vi "ProjG.vi"(8 "error in":errorcluster) -> (0 "error out":errorcluster)   [LabVIEW 2025]
uses:
  Enum(ctrl1).ctl
  Cluster(ctrl2).ctl
  Ldbrd_cl(ctrl3).ctl
  f9678b56-3cec-4690-80ba-5264990e7274.vi
  <vilib>/Array/Sort 2D Array - Pop Stack.vi
  <vilib>/Array/Sort 2D Array - Push Stack.vi
  <vilib>/Utility/file.llb/Read Delimited Spreadsheet (string).vi
  <vilib>/Instr/_visa.llb/VISA Configure Serial Port (Instr).vi
  <vilib>/Utility/file.llb/Write Delimited Spreadsheet (string).vi
  <vilib>/Analysis/NI_AAL_SigProc.lvlib
  <vilib>/ptbypt/NI_PtbyPt.lvlib
panel:
  in  "stop":bool
  out "LeaderBoard":string[][](array[string])
  in  "VISA port":refnum<visa-resource-name>
  out "HR":cluster{i32[], i32[]}(graph)
  out "Live HR":i32(graph)
  in  "Ldbrd":bool
  in  "Save":bool
  in  "Play":bool
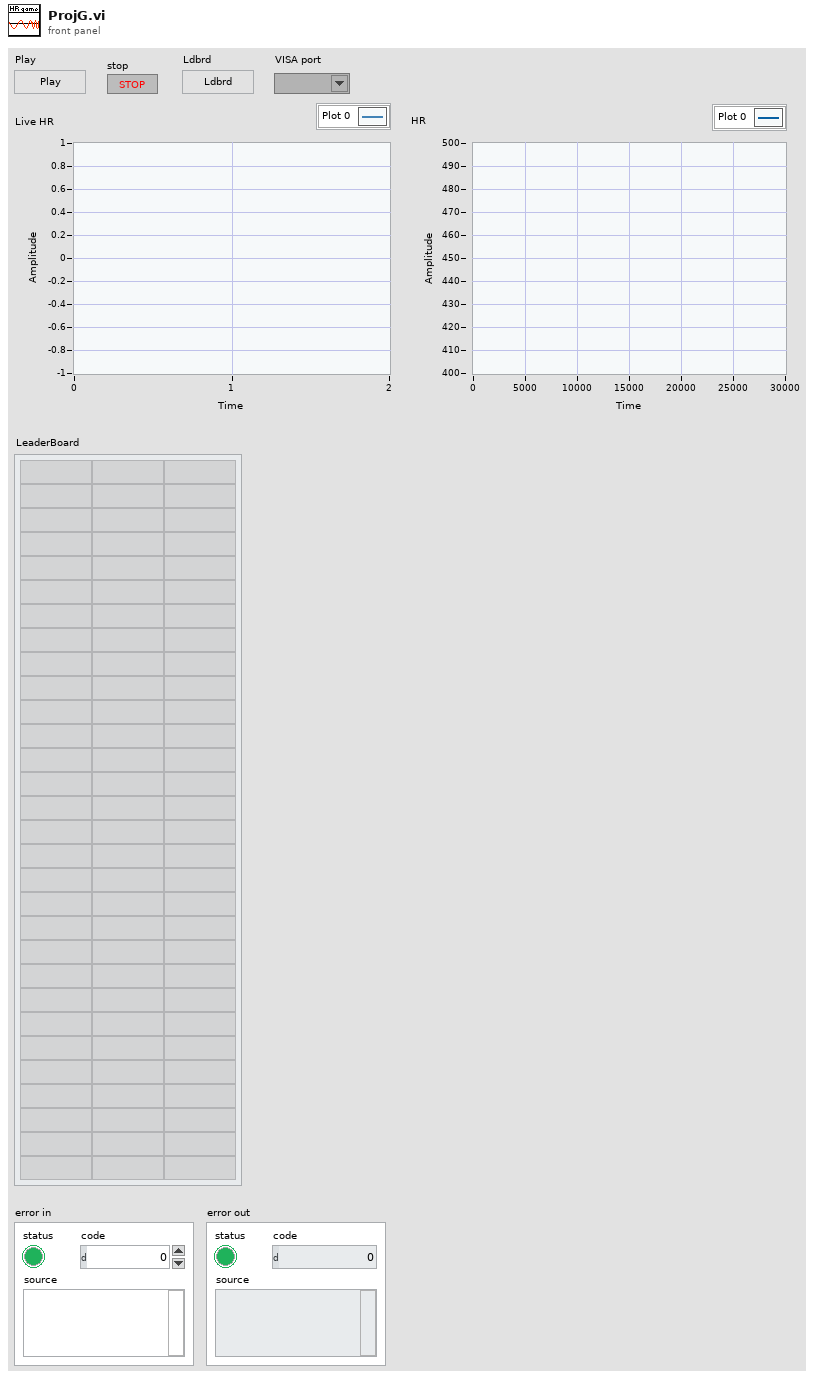
[diagram p1: front panel]
types:
  T1 = typedef "Ldbrd_cl(ctrl3).ctl" = cluster{"Ldbrd":string[][]}
  T2 = typedef "Cluster(ctrl2).ctl" = cluster{"Max HR":i8, "Name":string, "Avg HR":i8}
  T3 = typedef "Enum(ctrl1).ctl" = enum16{"Idle", "Init", "Play", "Ldbrd", "Display", "Save"}
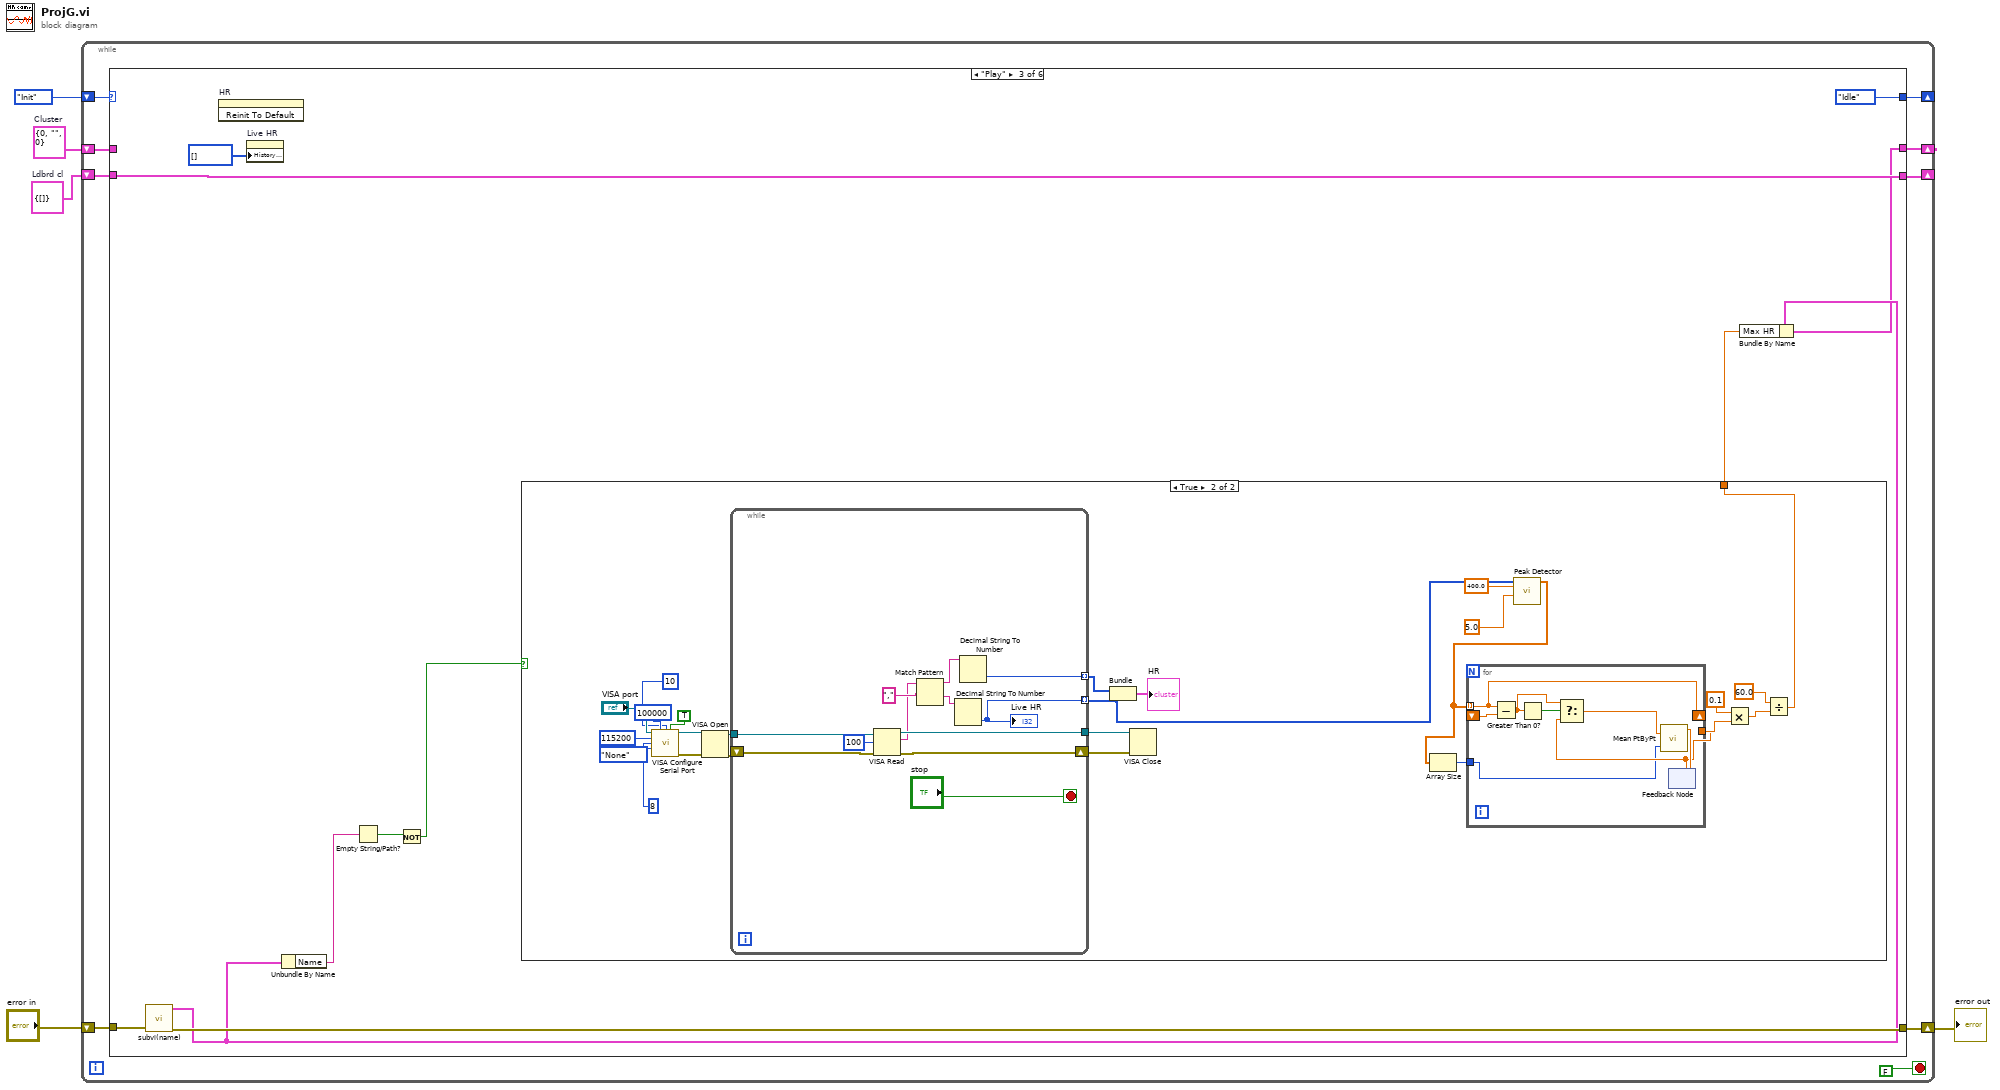
[diagram p0: block diagram]
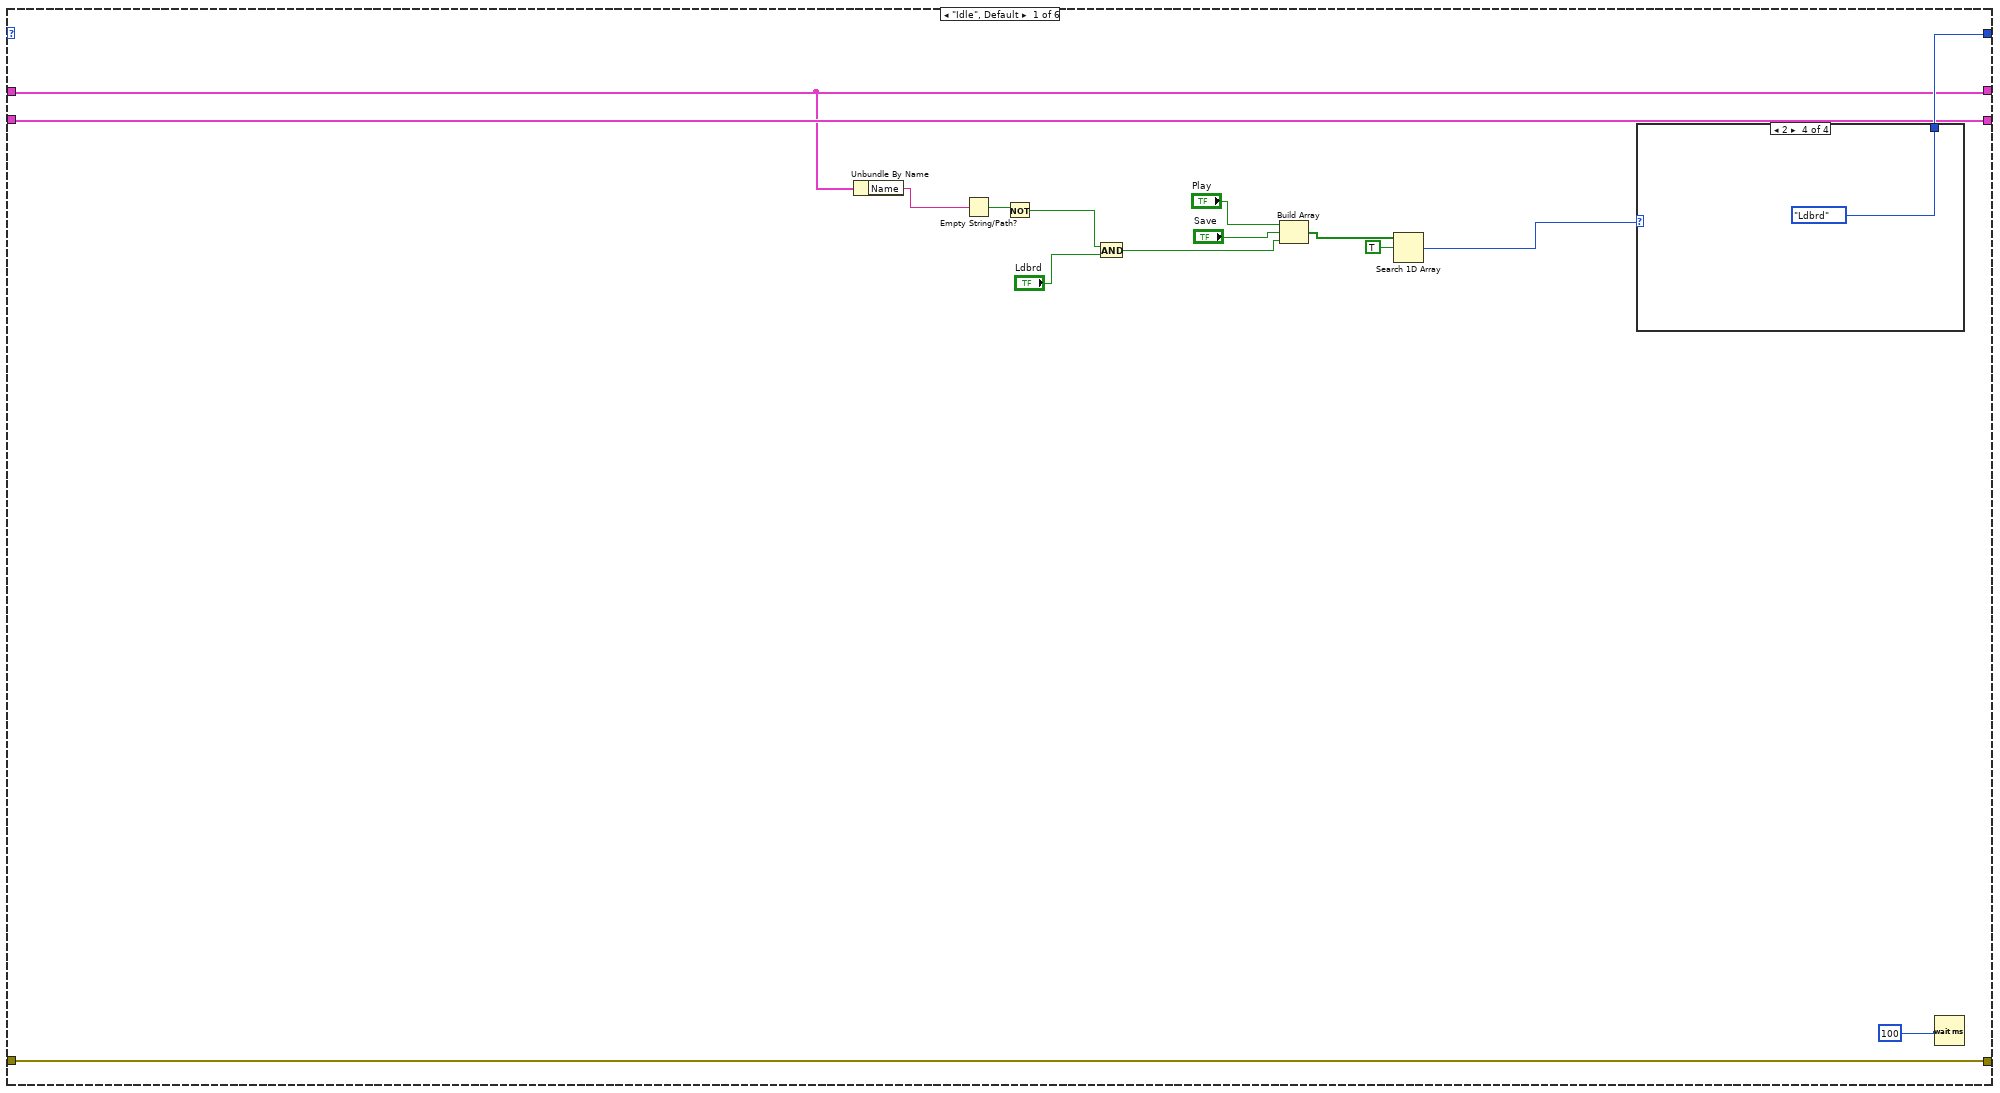
[diagram p2: hidden frame]
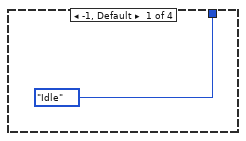
[diagram p3: hidden frame]
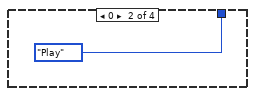
[diagram p4: hidden frame]
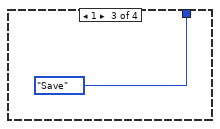
[diagram p5: hidden frame]
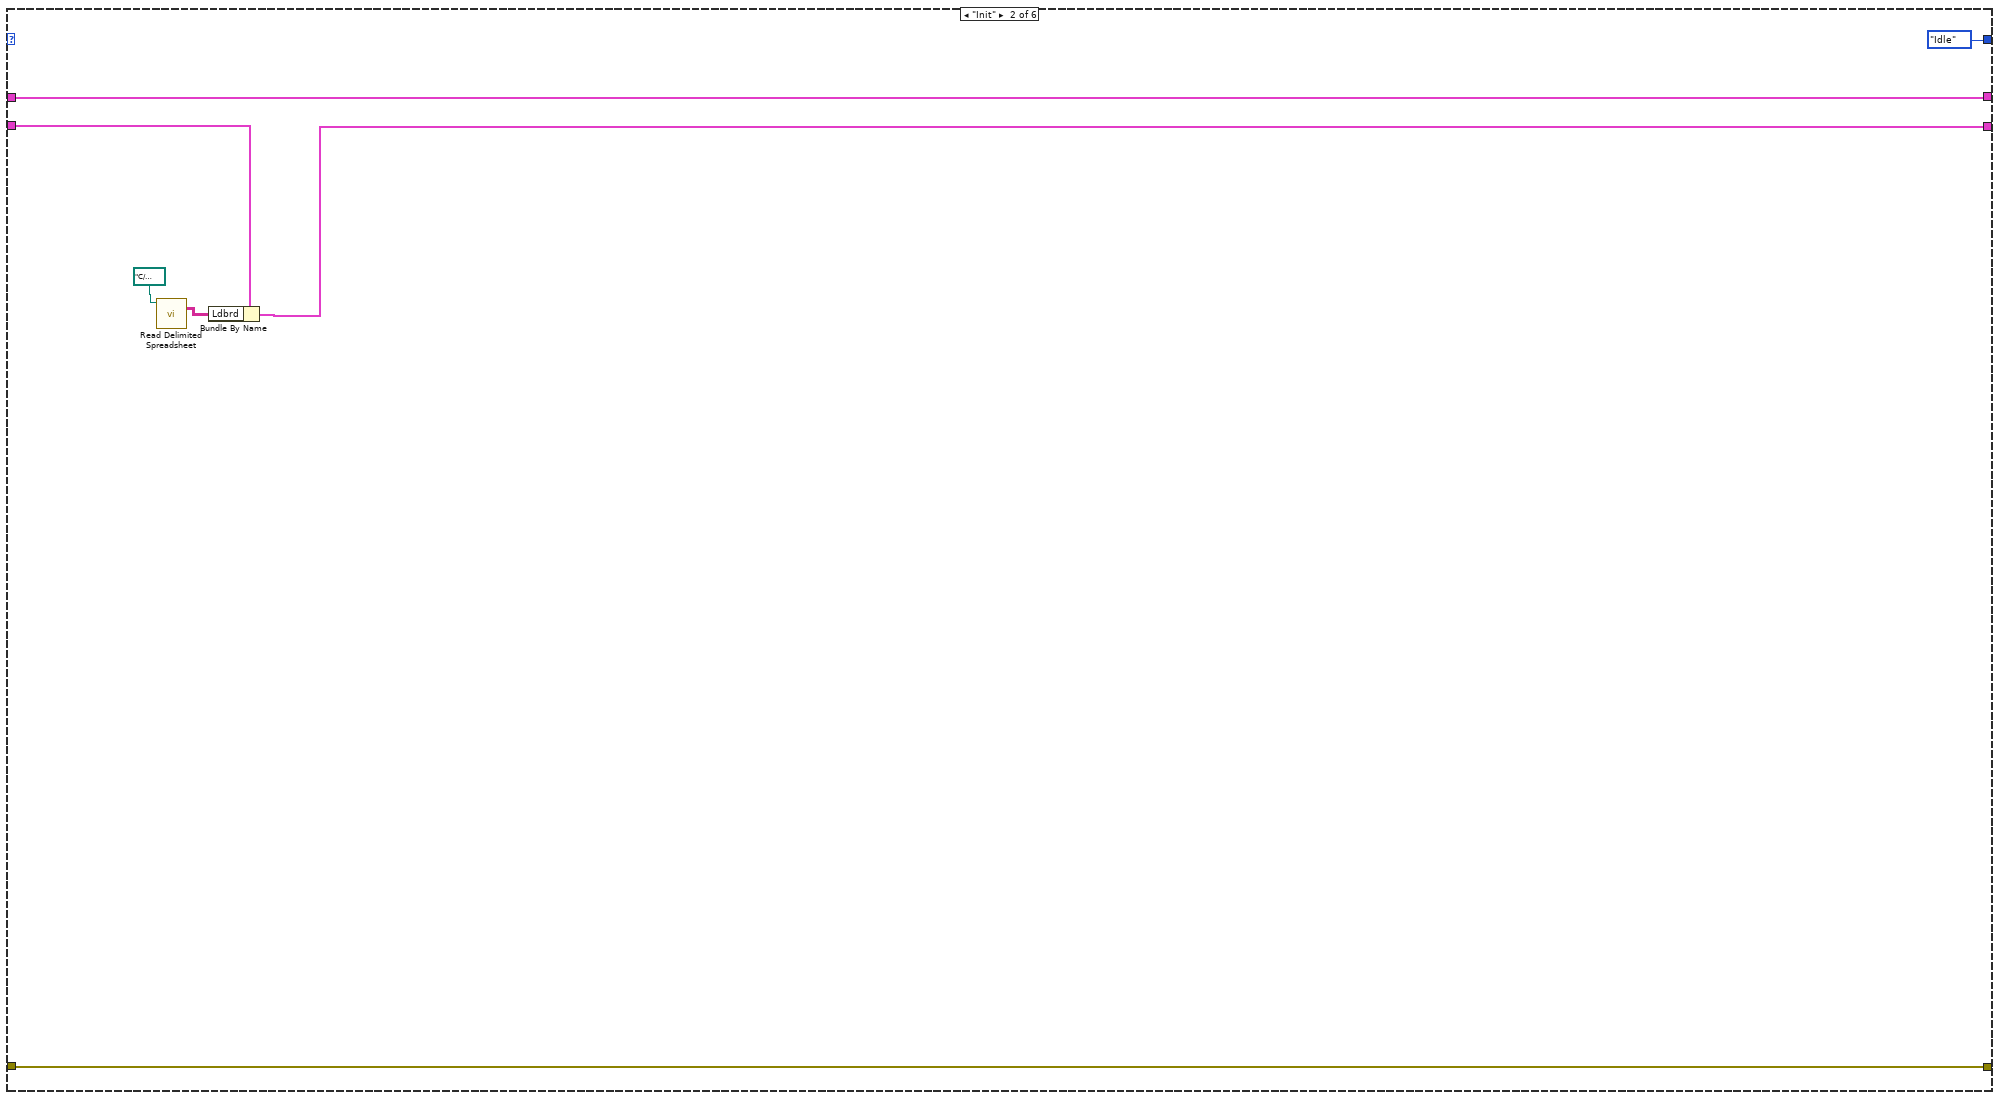
[diagram p6: hidden frame]
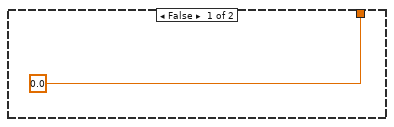
[diagram p7: hidden frame]
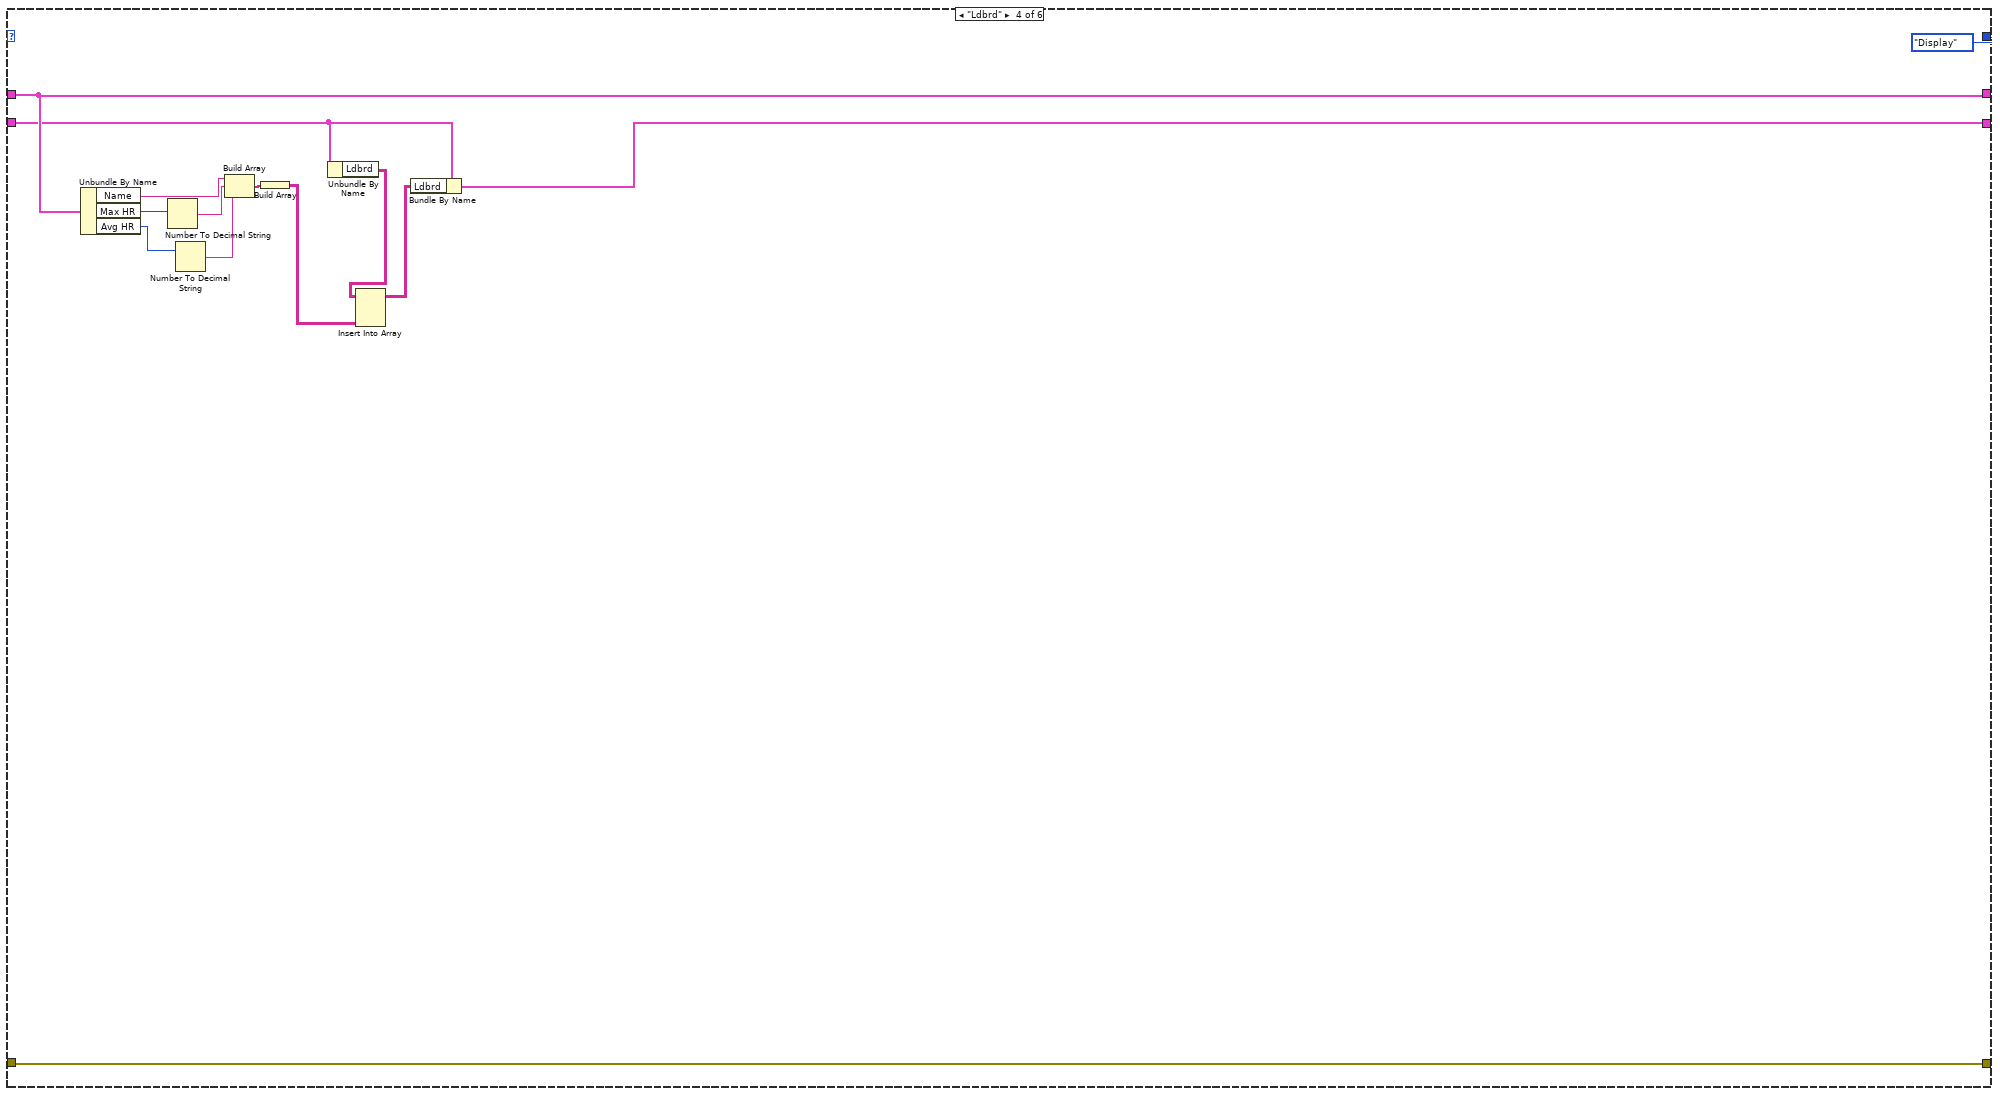
[diagram p8: hidden frame]
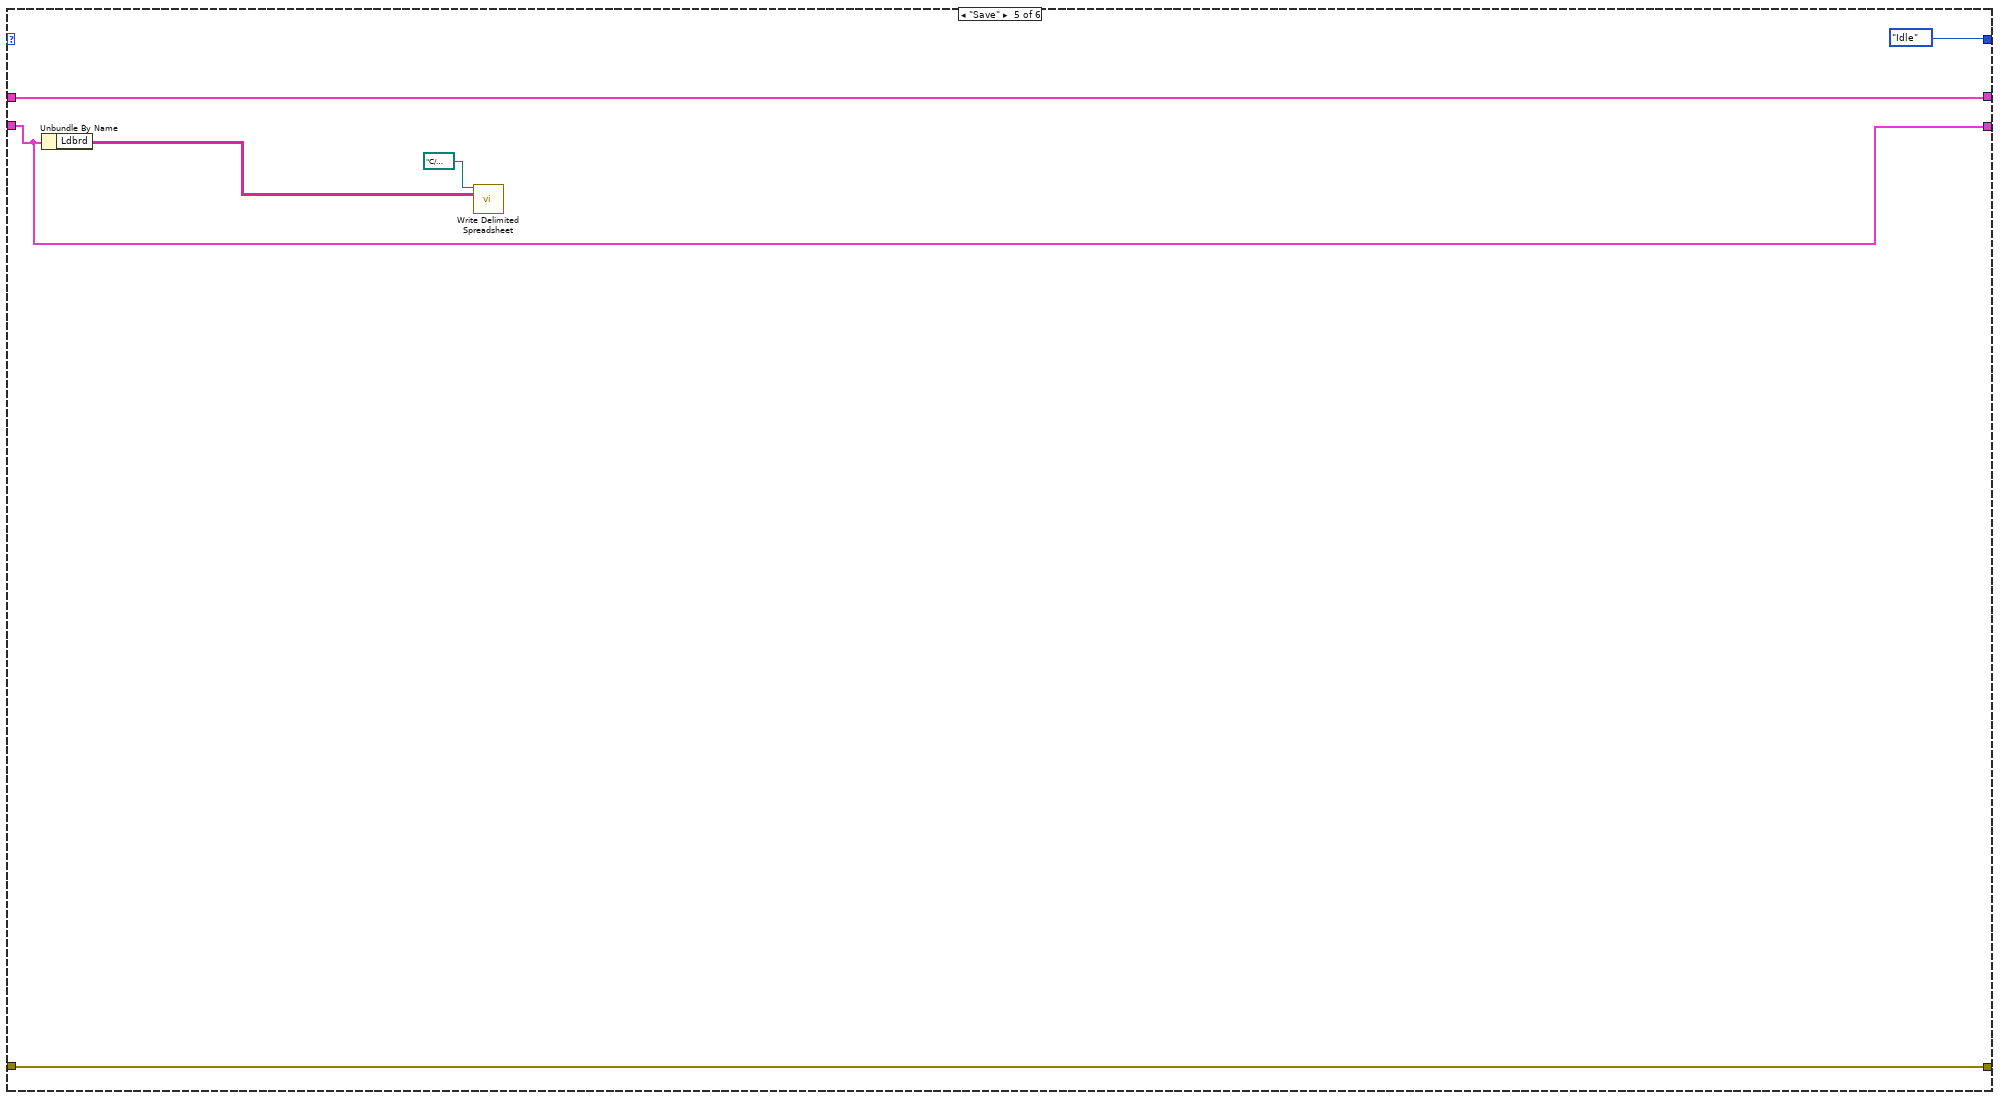
[diagram p9: hidden frame]
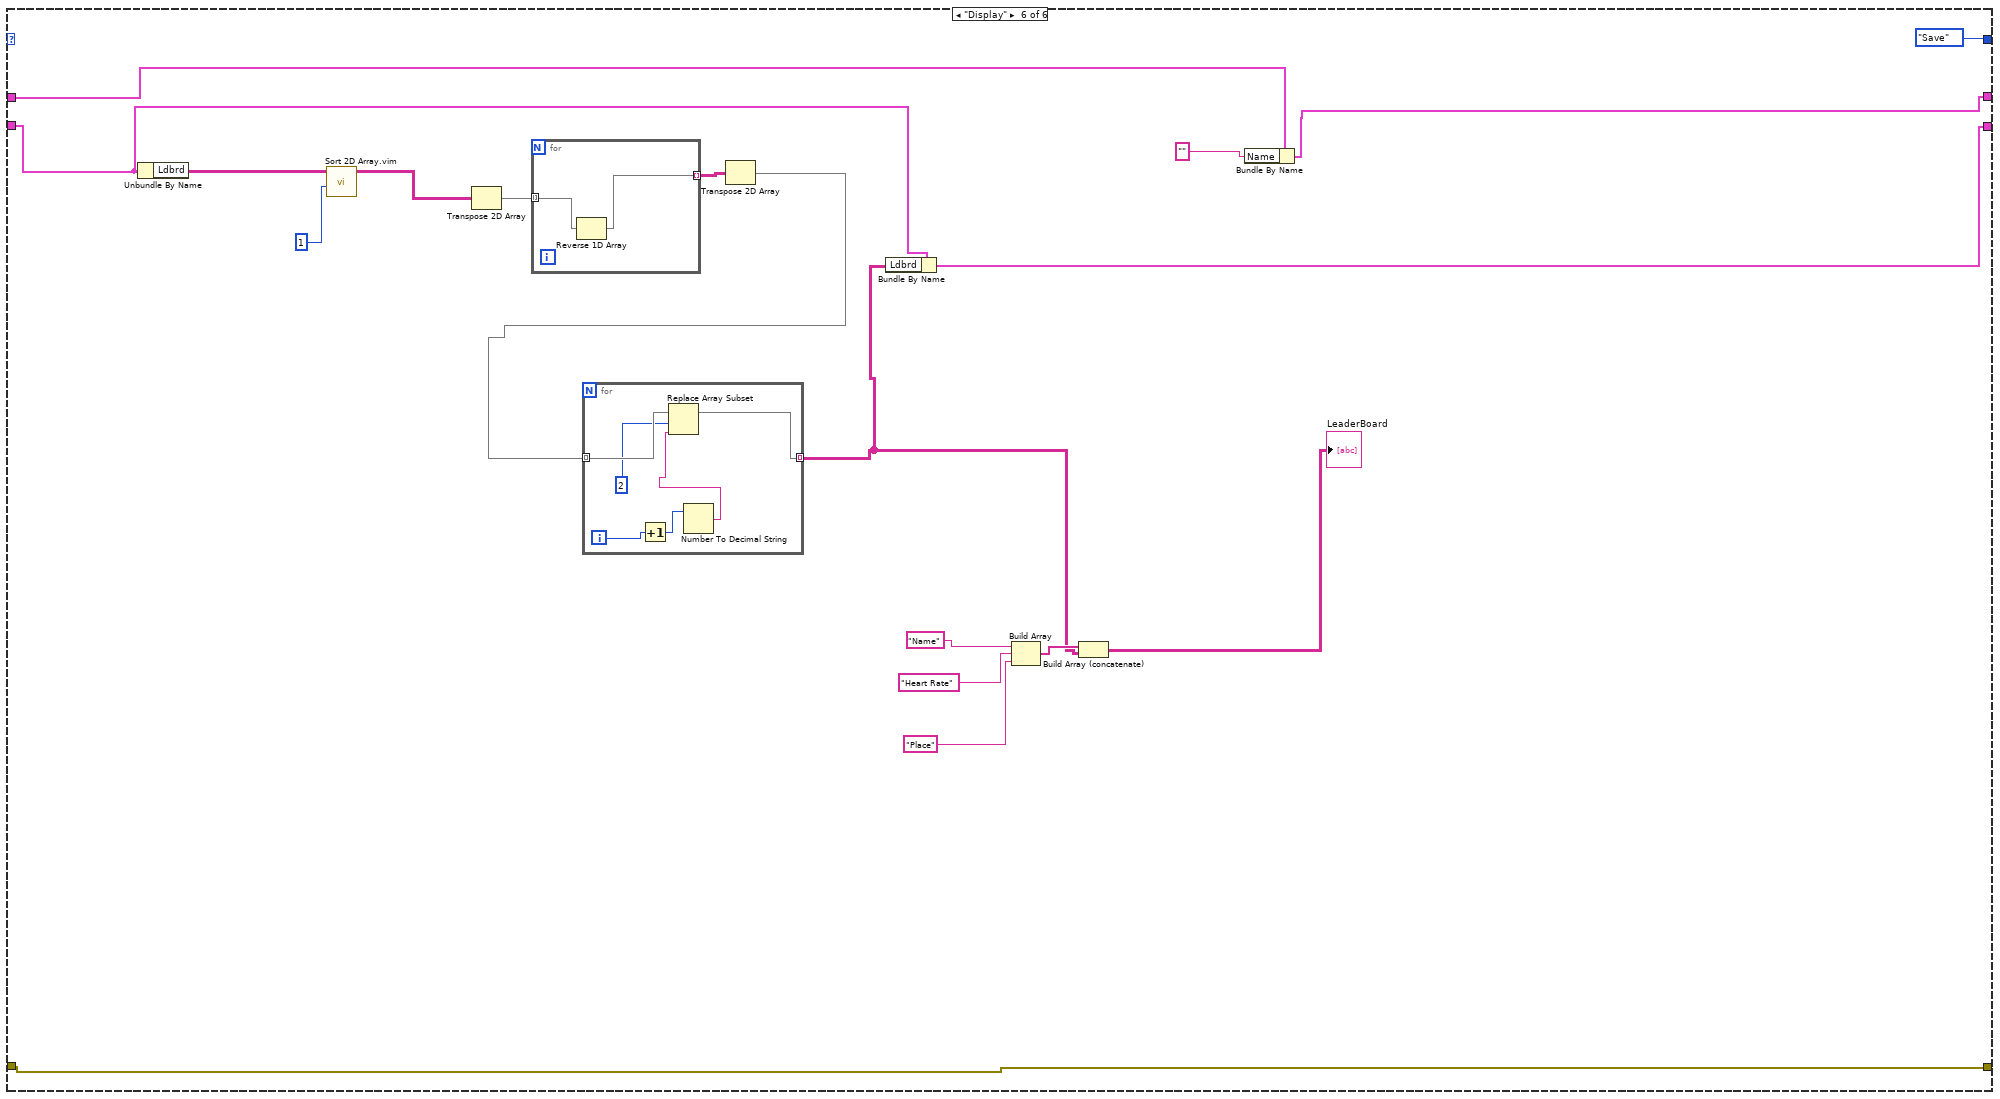
[diagram p10: hidden frame]
diagram:
  w1 = T1 {"Ldbrd"=[]}  # Ldbrd cl
  w2 = T2 {"Max HR"=0, "Name"="", "Avg HR"=0}  # Cluster
  n1 = while {
    shift-right: [w11] -> w4
    shift-left: "error in" -> [w12]
    shift-right: [w10] -> _
    shift-left: Enum(ctrl1)."Init" -> [w13]
    shift-right: [w8] -> _
    shift-left: w2 -> [w9]
    shift-right: [w7] -> _
    shift-left: w1 -> [w6]
    stop <- FALSE stop-if-true
    n2 = case shown="\"Play\"" w13 {
      tunnel: w12 -> [w29 w38 w51 w104 w112 w132]
      tunnel: [w29 w38 w50 w104 w112 w132] -> w11
      tunnel: [w22 Enum(ctrl1)."Idle" Enum(ctrl1)."Idle" Enum(ctrl1)."Display" Enum(ctrl1)."Idle" Enum(ctrl1)."Save"] -> w10
      tunnel: w9 -> [w20 w39 _ w107 w115 w119]
      tunnel: [w20 w39 w42 w107 w115 w118] -> w8
      tunnel: [w21 w34 w49 w106 w114 w134] -> w7
      tunnel: w6 -> [w21 w35 w49 w103 w114 w135]
      frame "Idle", Default {
        n3 = Unbundle By Name(w20) -> ("Name"=w19:string)
        n4 = Empty String/Path?(string/path=w19) -> (empty?=w18:bool)
        n5 = Not(x=w18) -> (.not. x?=w16:bool)
        n6 = And(x=w16, y="Ldbrd") -> (x .and. y?=w15:bool)
        n7 = Build Array("Play", "Save", w15) -> (w27:bool[])
        n8 = Search 1D Array(1D array=w27, element=TRUE) -> (index of element=w26:i32)  [unwired: 1 in]
        n9 = case shown="2" w26 {
          tunnel: [Enum(ctrl1)."Idle" Enum(ctrl1)."Play" Enum(ctrl1)."Save" Enum(ctrl1)."Ldbrd"] -> w22
          frame -1, Default {
          }
          frame 0 {
          }
          frame 1 {
          }
          frame 2 {
          }
        }
        n10 = Wait (ms)(milliseconds to wait=u32 100) -> ()  [unwired: 1 out]
      }
      frame "Init" {
        n11 = call-poly <vilib>:"Read Delimited Spreadsheet.vi"("file path (dialog if empty)"=path "C:/Users/micha/Desktop/AGH MTM/Semestr 3/Graficzne/Projekt/Ldbrd.txt") -> ("all rows"=w36:string[][])  [unwired: 9 in, 5 out]
        n12 = Bundle By Name(cluster=w35, "Ldbrd"=w36) -> (w34:T1)
      }
      frame "Play" {
        n13 = call "subvi(name).vi"("error in"=w51) -> ("error out"=w50:errorcluster, "Cluster ind"=w44:T2)  [unwired: 8 in, 1 out]
        n14 = invoke on="HR" class="XYGraph (strict)" method="Reinit To Default"() -> ()  [unwired: 3 in, 3 out]
        n15 = property on="Live HR" class="WFChart (strict)"("History Data"=i32[] []) -> ()  [unwired: 2 in, 2 out]
        n16 = Unbundle By Name(w44) -> ("Name"=w47:string)
        n17 = Empty String/Path?(string/path=w47) -> (empty?=w46:bool)
        n18 = Not(x=w46) -> (.not. x?=w45:bool)
        n19 = case shown="True" w45 {
          tunnel: [0.0 w59] -> w43
          frame False {
          }
          frame True {
            n20 = call-poly "VISA Configure Serial Port"("VISA resource name"="VISA port", "timeout (10sec)"=u32 100000, "termination char\n(0xA = '\\n' = LF)"=u8 10 ("termination char\n(0xA = '\\n' = LF)"), "Enable Termination\nChar (T)"=TRUE ("Enable Termination\nChar (T)"), "baud rate (9600)"=u32 115200, "data bits (8)"=u16 8, "parity (0:none)"=enum16{"None", "Odd", "Even", "Mark", "Space"}."None") -> ("VISA resource name out"=w75:refnum<visa-resource-name>, "error out"=w77:errorcluster)  [unwired: 7 in]
            n21 = VISA Open(error in (no error)=w77, VISA resource name=w75) -> (VISA resource name=w74:refnum<visa-resource-name>, error out=w76:errorcluster)  [unwired: 3 in]
            n22 = while {
              shift-right: [w96] -> w57
              shift-left: w76 -> [w97]
              tunnel: w74 -> [w87]
              tunnel: [w88] -> w63 mode=indexing
              tunnel: [w91] -> w70 mode=indexing
              tunnel: [w90] -> w58
              stop <- "stop" stop-if-true
              n23 = VISA Read(VISA resource name=w87, byte count=u32 100, error in (no error)=w97) -> (VISA resource name out=w90:refnum<visa-resource-name>, read buffer=w89:string, error out=w96:errorcluster)  [unwired: 1 out]
              n24 = Match Pattern(string=w89, regular expression=",") -> (before substring=w92:string, after substring=w93:string)  [unwired: 1 in, 2 out]
              n25 = Decimal String To Number(string=w93) -> (number=w88:i32)  [unwired: 2 in, 1 out]
              "Live HR" <- w88
              n26 = Decimal String To Number(string=w92) -> (number=w91:i32)  [unwired: 2 in, 1 out]
            }
            n27 = Bundle(w70, w63) -> (→"HR":cluster{i32[], i32[]})  [unwired: 1 in]
            n28 = VISA Close(VISA resource name=w58, error in (no error)=w57) -> ()  [unwired: 1 out]
            n29 = call <vilib>:"Peak Detector.vi"("width"=5.0, "threshold"=400.0, "X"=w63) -> ("Locations"=w54:dbl[])  [unwired: 4 in, 4 out]
            n30 = Array Size(array=w54) -> (size(s)=w55:i32)
            n31 = for {
              tunnel: w54 -> [w84] mode=indexing
              tunnel: [w79] -> w56
              shift-right: [w84] -> _
              shift-left: _ -> [w85]
              tunnel: w55 -> [w78]
              n32 = Subtract(x=w84, y=w85) -> (x-y=w81:dbl)
              n33 = Greater Than 0?(x=w81) -> (x > 0?=w83:bool)
              n34 = feedback #1() -> (w79:dbl)  [unwired: 1 in]
              n35 = Select(t=w81, s=w83, f=w79) -> (s? t:f=w82:dbl)
              n36 = call <vilib>:"Mean PtByPt.vi"("x"=w82, "sample length"=w78) -> ("mean"=w80:dbl)  [unwired: 2 in, 1 out]
              n37 = feedback-in #1(w80) -> ()
            }
            n38 = Multiply(x=0.1, y=w56) -> (x*y=w61:dbl)
            n39 = Divide(x=60.0, y=w61) -> (x/y=w59:dbl)
          }
        }
        n40 = Bundle By Name(cluster=w44, "Max HR"=w43) -> (w42:T2)
      }
      frame "Ldbrd" {
        n41 = Unbundle By Name(w107) -> ("Name"=w110:string, "Max HR"=w111:i8, "Avg HR"=w99:i8)
        n42 = Number To Decimal String(number=w111) -> (decimal integer string=w109:string)  [unwired: 1 in]
        n43 = Number To Decimal String(number=w99) -> (decimal integer string=w98:string)  [unwired: 1 in]
        n44 = Build Array(w110, w109, w98) -> (w108:string[])
        n45 = Build Array(w108) -> (w101:string[][])
        n46 = Unbundle By Name(w103) -> ("Ldbrd"=w102:string[][])
        n47 = Insert Into Array(array=w102, new element=w101) -> (w100:string[][])  [unwired: 2 in]
        n48 = Bundle By Name(cluster=w103, "Ldbrd"=w100) -> (w106:T1)
      }
      frame "Save" {
        n49 = Unbundle By Name(w114) -> ("Ldbrd"=w116:string[][])
        n50 = call-poly <vilib>:"Write Delimited Spreadsheet.vi"("file path (dialog if empty)"=path "C:/Users/micha/Desktop/AGH MTM/Semestr 3/Graficzne/Projekt/Ldbrd.txt", "2D data"=w116) -> ()  [unwired: 12 in, 2 out]
      }
      frame "Display" {
        n51 = Unbundle By Name(w135) -> ("Ldbrd"=w136:string[][])
        n52 = call "Sort 2D Array.vim"("index"=1, "2D array"=w136) -> ("sorted 2D array"=w130:string[][])  [unwired: 8 in, 1 out]
        n53 = Transpose 2D Array(2D array=w130) -> (transposed array=w129:string[][])
        n54 = for {
          tunnel: w129 -> [w144] mode=indexing
          tunnel: [w143] -> w128 mode=indexing
          n55 = Reverse 1D Array(array=w144) -> (reversed array=w143:string[])
        }
        n56 = Transpose 2D Array(2D array=w128) -> (transposed array=w127:string[][])
        n57 = for {
          tunnel: w127 -> [w140] mode=indexing
          tunnel: [w138] -> w121 mode=indexing
          i -> [w142]
          n58 = Increment(x=w142) -> (x+1=w141:i32)
          n59 = Number To Decimal String(number=w141) -> (decimal integer string=w139:string)  [unwired: 1 in]
          n60 = Replace Array Subset(array=w140, new element=w139, index=2) -> (w138:string[])
        }
        n61 = Bundle By Name(cluster=w135, "Ldbrd"=w121) -> (w134:T1)
        n62 = Build Array("Name", "Heart Rate", "Place") -> (w126:string[])
        n63 = Build Array (concatenate)(w126, w121) -> (→"LeaderBoard":string[][])
        n64 = Bundle By Name(cluster=w119, "Name"="") -> (w118:T2)
      }
    }
  }
  "error out" <- w4
